vi "XY Sample Stage History Points Holder.vi"(2 "Actions":T1=enum."Read", 7 "(x, y) Points":dbl[](array[numeric])) -> (8 "History Points":cluster{dbl[], dbl[]})   [LabVIEW 2016]
uses:
  XY Sample Stage Controls/XY Sample Stage History Actions.ctl
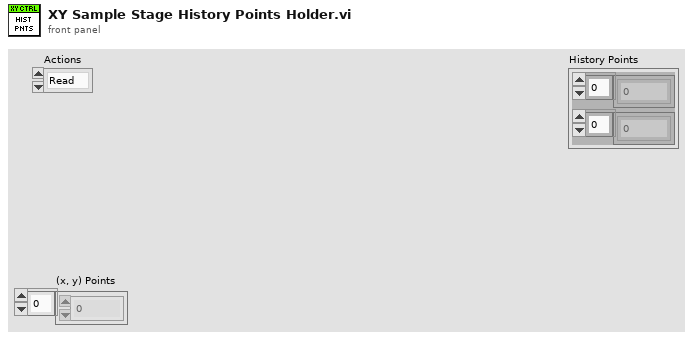
[diagram p1: front panel]
types:
  T1 = typedef "XY Sample Stage History Actions.ctl" = enum16{"Reset", "Write", "Read", "Set Zero"}
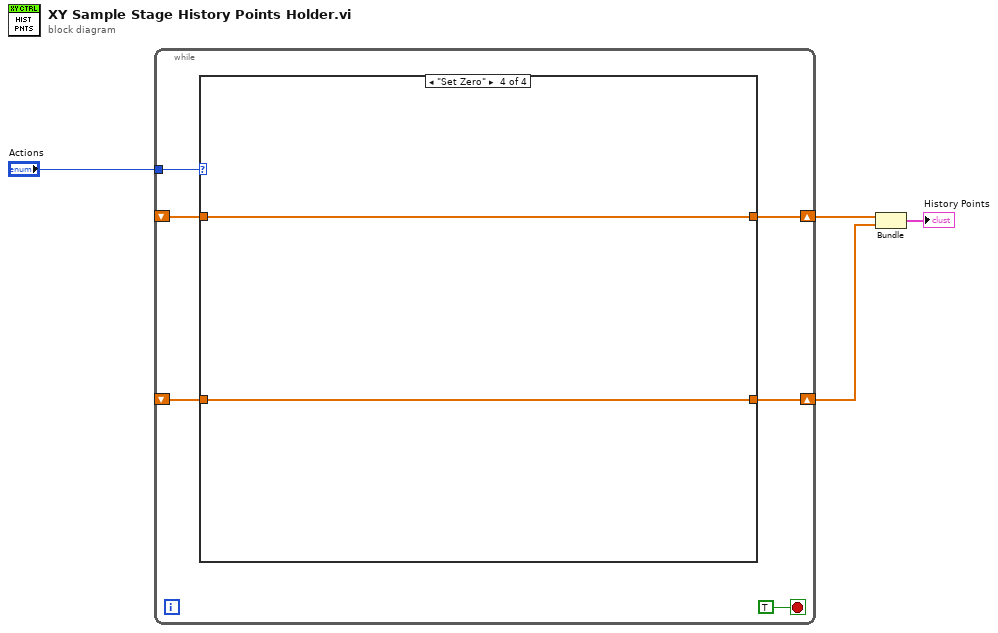
[diagram p0: block diagram]
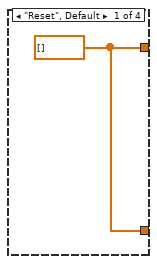
[diagram p2: hidden frame]
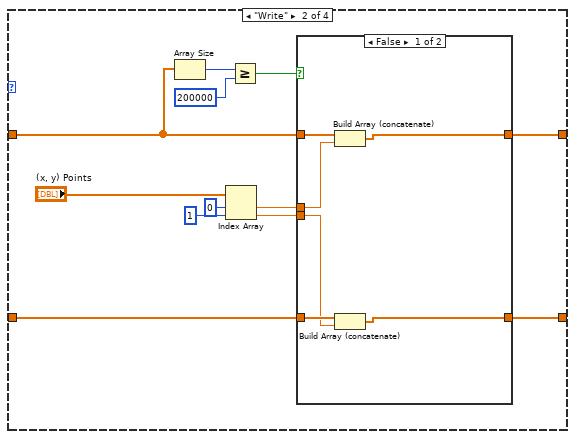
[diagram p3: hidden frame]
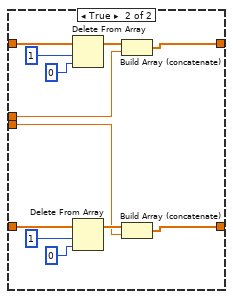
[diagram p4: hidden frame]
diagram:
  n1 = while {
    shift-right: [w8] -> w2
    shift-left: _ -> [w6]
    shift-right: [w7] -> w1
    shift-left: _ -> [w5]
    tunnel: "Actions" -> [w9]
    stop <- TRUE stop-if-true
    n2 = case shown="\"Set Zero\"" w9 {
      tunnel: [w11 w14 w43 w45] -> w8
      tunnel: [w11 w13 w42 w44] -> w7
      tunnel: w6 -> [_ w18 w43 w45]
      tunnel: w5 -> [_ w17 w42 w44]
      frame "Reset", Default {
        w11 = dbl[] []
      }
      frame "Write" {
        n3 = Array Size(array=w18) -> (size(s)=w23:i32)
        n4 = Index Array(array="(x, y) Points", index #1=0 ("index"), index #2=1 ("index")) -> (element #1=w16:dbl, element #2=w15:dbl)
        n5 = Greater Or Equal?(x=w23, y=200000) -> (x >= y?=w21:bool)
        n6 = case shown="False" w21 {
          tunnel: w18 -> [w29 w41]
          tunnel: w17 -> [w28 w36]
          tunnel: w16 -> [w26 w33]
          tunnel: w15 -> [w27 w32]
          tunnel: [w25 w31] -> w14
          tunnel: [w24 w30] -> w13
          frame False {
            n7 = Build Array (concatenate)(w29, w26) -> (w25:dbl[])
            n8 = Build Array (concatenate)(w28, w27) -> (w24:dbl[])
          }
          frame True {
            n9 = Delete From Array(array=w41, length=1, index=0 ("length")) -> (array with subset deleted=w35:dbl[])  [unwired: 1 out]
            n10 = Delete From Array(array=w36, length=1, index=0 ("length")) -> (array with subset deleted=w34:dbl[])  [unwired: 1 out]
            n11 = Build Array (concatenate)(w35, w33) -> (w31:dbl[])
            n12 = Build Array (concatenate)(w34, w32) -> (w30:dbl[])
          }
        }
      }
      frame "Read" {
      }
      frame "Set Zero" {
      }
    }
  }
  n13 = Bundle(w2, w1) -> (→"History Points":cluster{dbl[], dbl[]})  [unwired: 1 in]
